vi "CalcExpress - Get Error Message.vi"(6 "error in":bool, 9 "CE InstanceRef":T1) -> (0 "error out":bool, 1 "error description":string, 2 "error code":i32, 3 "dup CE InstanceRef":T1)   [LabVIEW 2021]
doc: "The VI returns information on an error if any occurred during parsing or evaluation of a script associated with the <B>CE InstanceRef</B>.\n\nFor more information, see help for this VI.\n\n::: CalcExpress Toolkit :::\nCopyright (c) 2000-2026 Konstantin Shifershteyn. All rights reserved."
uses:
  cetypes.llb/CalcExpress Instance RefNum.ctl
  cersrc/celveng32.dll
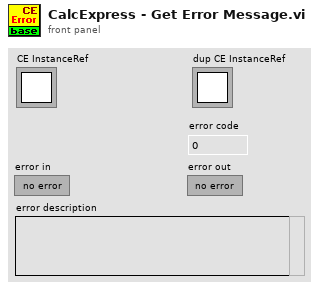
[diagram p1: front panel]
types:
  T1 = typedef "CalcExpress Instance RefNum.ctl" = refnum<k1>
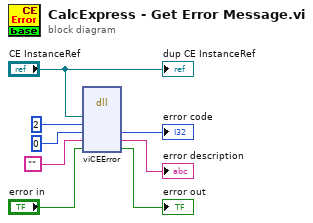
[diagram p0: block diagram]
diagram:
  n1 = dll-call lib="C:/LV Projects/CalcExpress 40 LV2021/vi.lib/addons/CalcExpress/cersrc/celveng*.dll" fn="viCEError"("iRef"="CE InstanceRef", "cmd"=2 ("get"), "errCode"=0, "erMsg"="", "erf"="error in") -> ("errCode"=→"error code":i32, "erMsg"=→"error description":string, "erf"=→"error out":bool)  [unwired: 6 in, 2 out]
  "dup CE InstanceRef" <- "CE InstanceRef"
